vi "Main.vi"(11 "Module Admin":refnum<class "Delacor_lib_QMH_Cloneable Module Admin.lvclass">) -> ()   [LabVIEW 2026, in "UserEventRecorder.lvlib"]
doc: "This template is based off of the Queued Message Handler design pattern and the Queued Message Handler project template that ships with LabVIEW.\n\nThe main difference is that the queue is private to this module and communication between modules is performed via Broadcast and Request events.\n\nRequest events are wrapped in public API methods and are handled in the Event Handling Loop (EHL) of this VI. Any module can register for Broadcast events sent by this module. The EHL generates messages based on user interface actions.\n\nThe Message Handling Loop (MHL) processes messages generated by the EHL, or by other messages. The messages are string values, so new messages can be added easily to the Message Cases case structure in the MHL. Each message cluster can also provide an optional value for Message Data, which is a variant that can be converted to whatever message-specific data is required.\n_____\nBased on DQMH Dev Tools: Project Template 7.1.2.1547."
uses:
  UserEventRecorder.lvlib
  <vilib>/Delacor/Delacor QMH/Libraries/Cloneable Module Admin_class/Delacor_lib_QMH_Cloneable Module Admin.lvclass
  TestEvent.ctl
  <vilib>/Wovalab/Utilities/Helper Loop Periodic Timing/Late Execution Mode--enum.ctl
  KeyboardAndMouseDataAcquisition.ctl
  <vilib>/Wovalab/Utilities/Helper Loop Periodic Timing/Helper Loop Periodic Timing.lvclass/Helper Loop Periodic Timing.ctl
  Module Data--cluster.ctl
  <vilib>/Delacor/Delacor QMH/Libraries/Cloneable Module Admin_class/Delacor_lib_QMH_Cloneable Module Admin.lvclass/Delacor_lib_QMH_Cloneable Module Admin.ctl
  Record Frame Mouse Metadata Argument--cluster.ctl
  <vilib>/Delacor/Delacor QMH/Libraries/Message Queue_class/Delacor_lib_QMH_Message Queue.lvclass/Delacor_lib_QMH_Message Queue.ctl
  Stop Argument--cluster.ctl
  <vilib>/Delacor/Delacor QMH/Libraries/Module Admin_class/Delacor_lib_QMH_Module Admin.lvclass/Delacor_lib_QMH_Module Admin.ctl
  <vilib>/Utility/miscctls.llb/LVPointTypeDef.ctl
  6b0c7d21-e3a6-4e04-8aec-f5c565291270.vi
  7c070138-7b6f-4615-b0c4-f77ec53dd64e.vi
  <vilib>/Delacor/Delacor QMH/Libraries/Cloneable Module Admin_class/Delacor_lib_QMH_Get Module ID.vi
  <vilib>/Wovalab/Utilities/Helper Loop Periodic Timing/Read Current Number Of Execution.vi
  <vilib>/Delacor/Delacor QMH/Libraries/Message Queue_class/Delacor_lib_QMH_Enqueue Message (Single).vi
  <vilib>/Delacor/Delacor QMH/Libraries/Module Admin_class/Delacor_lib_QMH_Get External Launch.vi
  <vilib>/Wovalab/Utilities/Helper Loop Periodic Timing/Stop Helper Loop Internal.vi
  <vilib>/Wovalab/Utilities/Helper Loop Periodic Timing/U32 Max Value--constant.vi
  <vilib>/Wovalab/Utilities/Helper Loop Periodic Timing/Update Last Execution Time.vi
  <vilib>/Wovalab/Utilities/Helper Loop Periodic Timing/Loops Events AE.vi
  <vilib>/Wovalab/Utilities/Helper Loop Periodic Timing/Notify Monitoring Window.vi
  <vilib>/Wovalab/Utilities/Helper Loop Periodic Timing/Monitoring--global.vi
  Core/global.vi
  <userlib>/_OpenG.lib/comparison/comparison.llb/String Changed__ogtk.vi
  <vilib>/Utility/inputDevices.llb/mouseAcquire.vi
  <vilib>/Utility/inputDevices.llb/keyboardAcquire.vi
  <vilib>/JDP Science/JSONtext/Variant to JSON Text.vi
  <vilib>/Utility/inputDevices.llb/closeMouse.vi
  <vilib>/Utility/inputDevices.llb/closeKeyboard.vi
  <vilib>/Wovalab/Utilities/Helper Loop Periodic Timing/Helper Loop Periodic Timing.lvclass
  <vilib>/JDP Science/JSONtext/LVClass Serializer/JSONtext LVClass Serializer.lvclass
  <vilib>/Delacor/Delacor QMH/Libraries/Message Queue_class/Delacor_lib_QMH_Message Queue.lvclass
  Launcher/Launcher.lvlib
  Core/Core.lvlib
  <userlib>/_OpenG.lib/comparison/comparison.llb/openg_comparison__ogtk.lvlib
panel:
  out "TestEvent":T1
  out "axis info":T2
  out "button info":T3
  out "keys pressed":T4(array[ring])
  out "error out":errorcluster
  out "Status":string
  in  "Simulate EHL Error":bool
  in  "Simulate MHL Error":bool
  # "Other processes communicate with this Module via its Public API (wrappers for its Request Events).\n\nThis Module communicates with other processes via its Broadcast Events.\nAny process that wants to receive these messages can register for this module's Broadcast events."
  # "This template is for the DQMH framework. See the block diagram for more information on how to use this template."
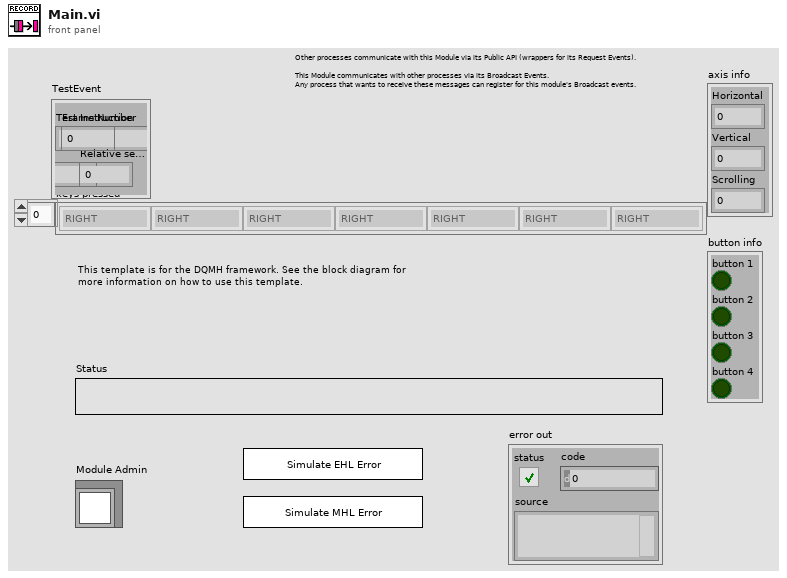
[diagram p1: front panel]
types:
  T1 = typedef "TestEvent.ctl" = cluster{"Test Instruction":string, "Sample Number":u32, "Relative seconds":dbl, "Frame Number":u32}
  T2 = cluster{"Horizontal":i32, "Vertical":i32, "Scrolling":i32}
  T3 = cluster{"button 1":bool, "button 2":bool, "button 3":bool, "button 4":bool}
  T4 = enum16{"0", "1", "2", "3", "4", "5", "6", "7", "8", "9", "A", "B", "C", "D", "E", "F", "G", "H", "I", "J", "K", "L", "M", "N", "O", "P", "Q", "R", "S", "T", "U", "V", "W", "X", "Y", "Z", "F1", "F2", "F3", "F4", "F5", "F6", "F7", "F8", "F9", "F10", "F11", "F12", "F13", "F14", "F15", "ADD", "BACK", "BACKSLASH", "CAPITAL", "COMMA", "DECIMAL", "DELETE", "DIVIDE", "DOWN", "END", "EQUALS", "ESCAPE", "GRAVE (`)", "HOME", "INSERT", "LBRACKET", "LCONTROL", "LEFT", "L ALT", "LSHIFT", "LWIN", "MINUS", "MULTIPLY", "NEXT", "NUMLOCK", "NUMPAD_0", "NUMPAD_1", "NUMPAD_2", "NUMPAD_3", "NUMPAD_4", "NUMPAD_5", "NUMPAD_6", "NUMPAD_7", "NUMPAD_8", "NUMPAD_9", "PAUSE", "PERIOD", "PRIOR (PG UP)", "RBRACKET", "RCONTROL", "RETURN", "RIGHT", "R ALT", "RSHIFT", "RWIN", "SCROLL", "SEMICOLON", "SLASH", "SPACE", "SUBTRACT", "TAB", "UP", "ENTER (num pad)", "' (quote)"}[]
  T5 = typedef "KeyboardAndMouseDataAcquisition.ctl" = cluster{"axis info":cluster{"Horizontal":i32, "Vertical":i32, "Scrolling":i32}, "button info":cluster{"button 1":bool, "button 2":bool, "button 3":bool, "button 4":bool}, "Relative Time (User Event)":dbl, "Sample Number":u32, "Relative Time (Frame 0)":dbl, "key mode":enum16{"RELATIVE", "ABSOLUTE"}, "Frame Number":u32, "Keyboard Key Pressed":enum16{"0", "1", "2", "3", "4", "5", "6", "7", "8", "9", "A", "B", "C", "D", "E", "F", "G", "H", "I", "J", "K", "L", "M", "N", "O", "P", "Q", "R", "S", "T", "U", "V", "W", "X", "Y", "Z", "F1", "F2", "F3", "F4", "F5", "F6", "F7", "F8", "F9", "F10", "F11", "F12", "F13", "F14", "F15", "ADD", "BACK", "BACKSLASH", "CAPITAL", "COMMA", "DECIMAL", "DELETE", "DIVIDE", "DOWN", "END", "EQUALS", "ESCAPE", "GRAVE (`)", "HOME", "INSERT", "LBRACKET", "LCONTROL", "LEFT", "L ALT", "LSHIFT", "LWIN", "MINUS", "MULTIPLY", "NEXT", "NUMLOCK", "NUMPAD_0", "NUMPAD_1", "NUMPAD_2", "NUMPAD_3", "NUMPAD_4", "NUMPAD_5", "NUMPAD_6", "NUMPAD_7", "NUMPAD_8", "NUMPAD_9", "PAUSE", "PERIOD", "PRIOR (PG UP)", "RBRACKET", "RCONTROL", "RETURN", "RIGHT", "R ALT", "RSHIFT", "RWIN", "SCROLL", "SEMICOLON", "SLASH", "SPACE", "SUBTRACT", "TAB", "UP", "ENTER (num pad)", "' (quote)"}, "Keyboard No Op":bool}
  T6 = typedef "Wovalab_lib_Utilities.lvlib/Helper Loop Periodic Timing.lvclass/Late Execution Mode--enum.ctl" = enum16{"No change", "Process missed periods ignoring original phase", "Process missed periods maintaining original phase"}
  T7 = typedef "UserEventRecorder.lvlib/Request Events--cluster.ctl" = cluster{"Stop Module":refnum<user-event>, "Show Panel":refnum<user-event>, "Hide Panel":refnum<user-event>, "Show Diagram":refnum<user-event>, "Get Module Execution Status":refnum<user-event>, "Record Frame Mouse Metadata":refnum<user-event>, "Local Instance":T8}
  T8 = typedef "UserEventRecorder.lvlib/Local Instance Request Events--cluster.ctl" = cluster{"Test Event Triggered":refnum<user-event>}
  T9 = typedef "Launcher.lvlib/Broadcast Events--cluster.ctl" = cluster{"Module Did Init":refnum<user-event>, "Status Updated":refnum<user-event>, "Error Reported":refnum<user-event>, "Module Did Stop":refnum<user-event>, "Update Module Execution Status":refnum<user-event>, "Start Capture Detection Loop":refnum<user-event>, "Benchmark Started":refnum<user-event>, "Broadcast number of frames and run ID":refnum<user-event>}
  T10 = typedef "UserEventRecorder.lvlib/Module Data--cluster.ctl" = cluster{"Status":string}
  T11 = enum16{"0", "1", "2", "3", "4", "5", "6", "7", "8", "9", "A", "B", "C", "D", "E", "F", "G", "H", "I", "J", "K", "L", "M", "N", "O", "P", "Q", "R", "S", "T", "U", "V", "W", "X", "Y", "Z", "F1", "F2", "F3", "F4", "F5", "F6", "F7", "F8", "F9", "F10", "F11", "F12", "F13", "F14", "F15", "ADD", "BACK", "BACKSLASH", "CAPITAL", "COMMA", "DECIMAL", "DELETE", "DIVIDE", "DOWN", "END", "EQUALS", "ESCAPE", "GRAVE (`)", "HOME", "INSERT", "LBRACKET", "LCONTROL", "LEFT", "L ALT", "LSHIFT", "LWIN", "MINUS", "MULTIPLY", "NEXT", "NUMLOCK", "NUMPAD_0", "NUMPAD_1", "NUMPAD_2", "NUMPAD_3", "NUMPAD_4", "NUMPAD_5", "NUMPAD_6", "NUMPAD_7", "NUMPAD_8", "NUMPAD_9", "PAUSE", "PERIOD", "PRIOR (PG UP)", "RBRACKET", "RCONTROL", "RETURN", "RIGHT", "R ALT", "RSHIFT", "RWIN", "SCROLL", "SEMICOLON", "SLASH", "SPACE", "SUBTRACT", "TAB", "UP", "ENTER (num pad)", "' (quote)"}
  T12 = enum32{"invalid lock state", "Not Locked", "Locked (No Password)", "Password-protected"}
  T13 = typedef "UserEventRecorder.lvlib/Stop Argument--cluster.ctl" = cluster{"Module ID":i32, "Origin":string, "Exit via Stop Module Req?":bool, "Wait for Module to stop?":bool}
  T14 = typedef "LVPointTypeDef.ctl" = cluster{"Horizontal":i16, "Vertical":i16}
  T15 = enum32{"Invalid", "Standard", "Closed", "Hidden", "Minimized", "Maximized"}
  T16 = typedef "UserEventRecorder.lvlib/Record Frame Mouse Metadata Argument--cluster.ctl" = cluster{"Module ID":i32, "KeyboardAndMouseData":T5}
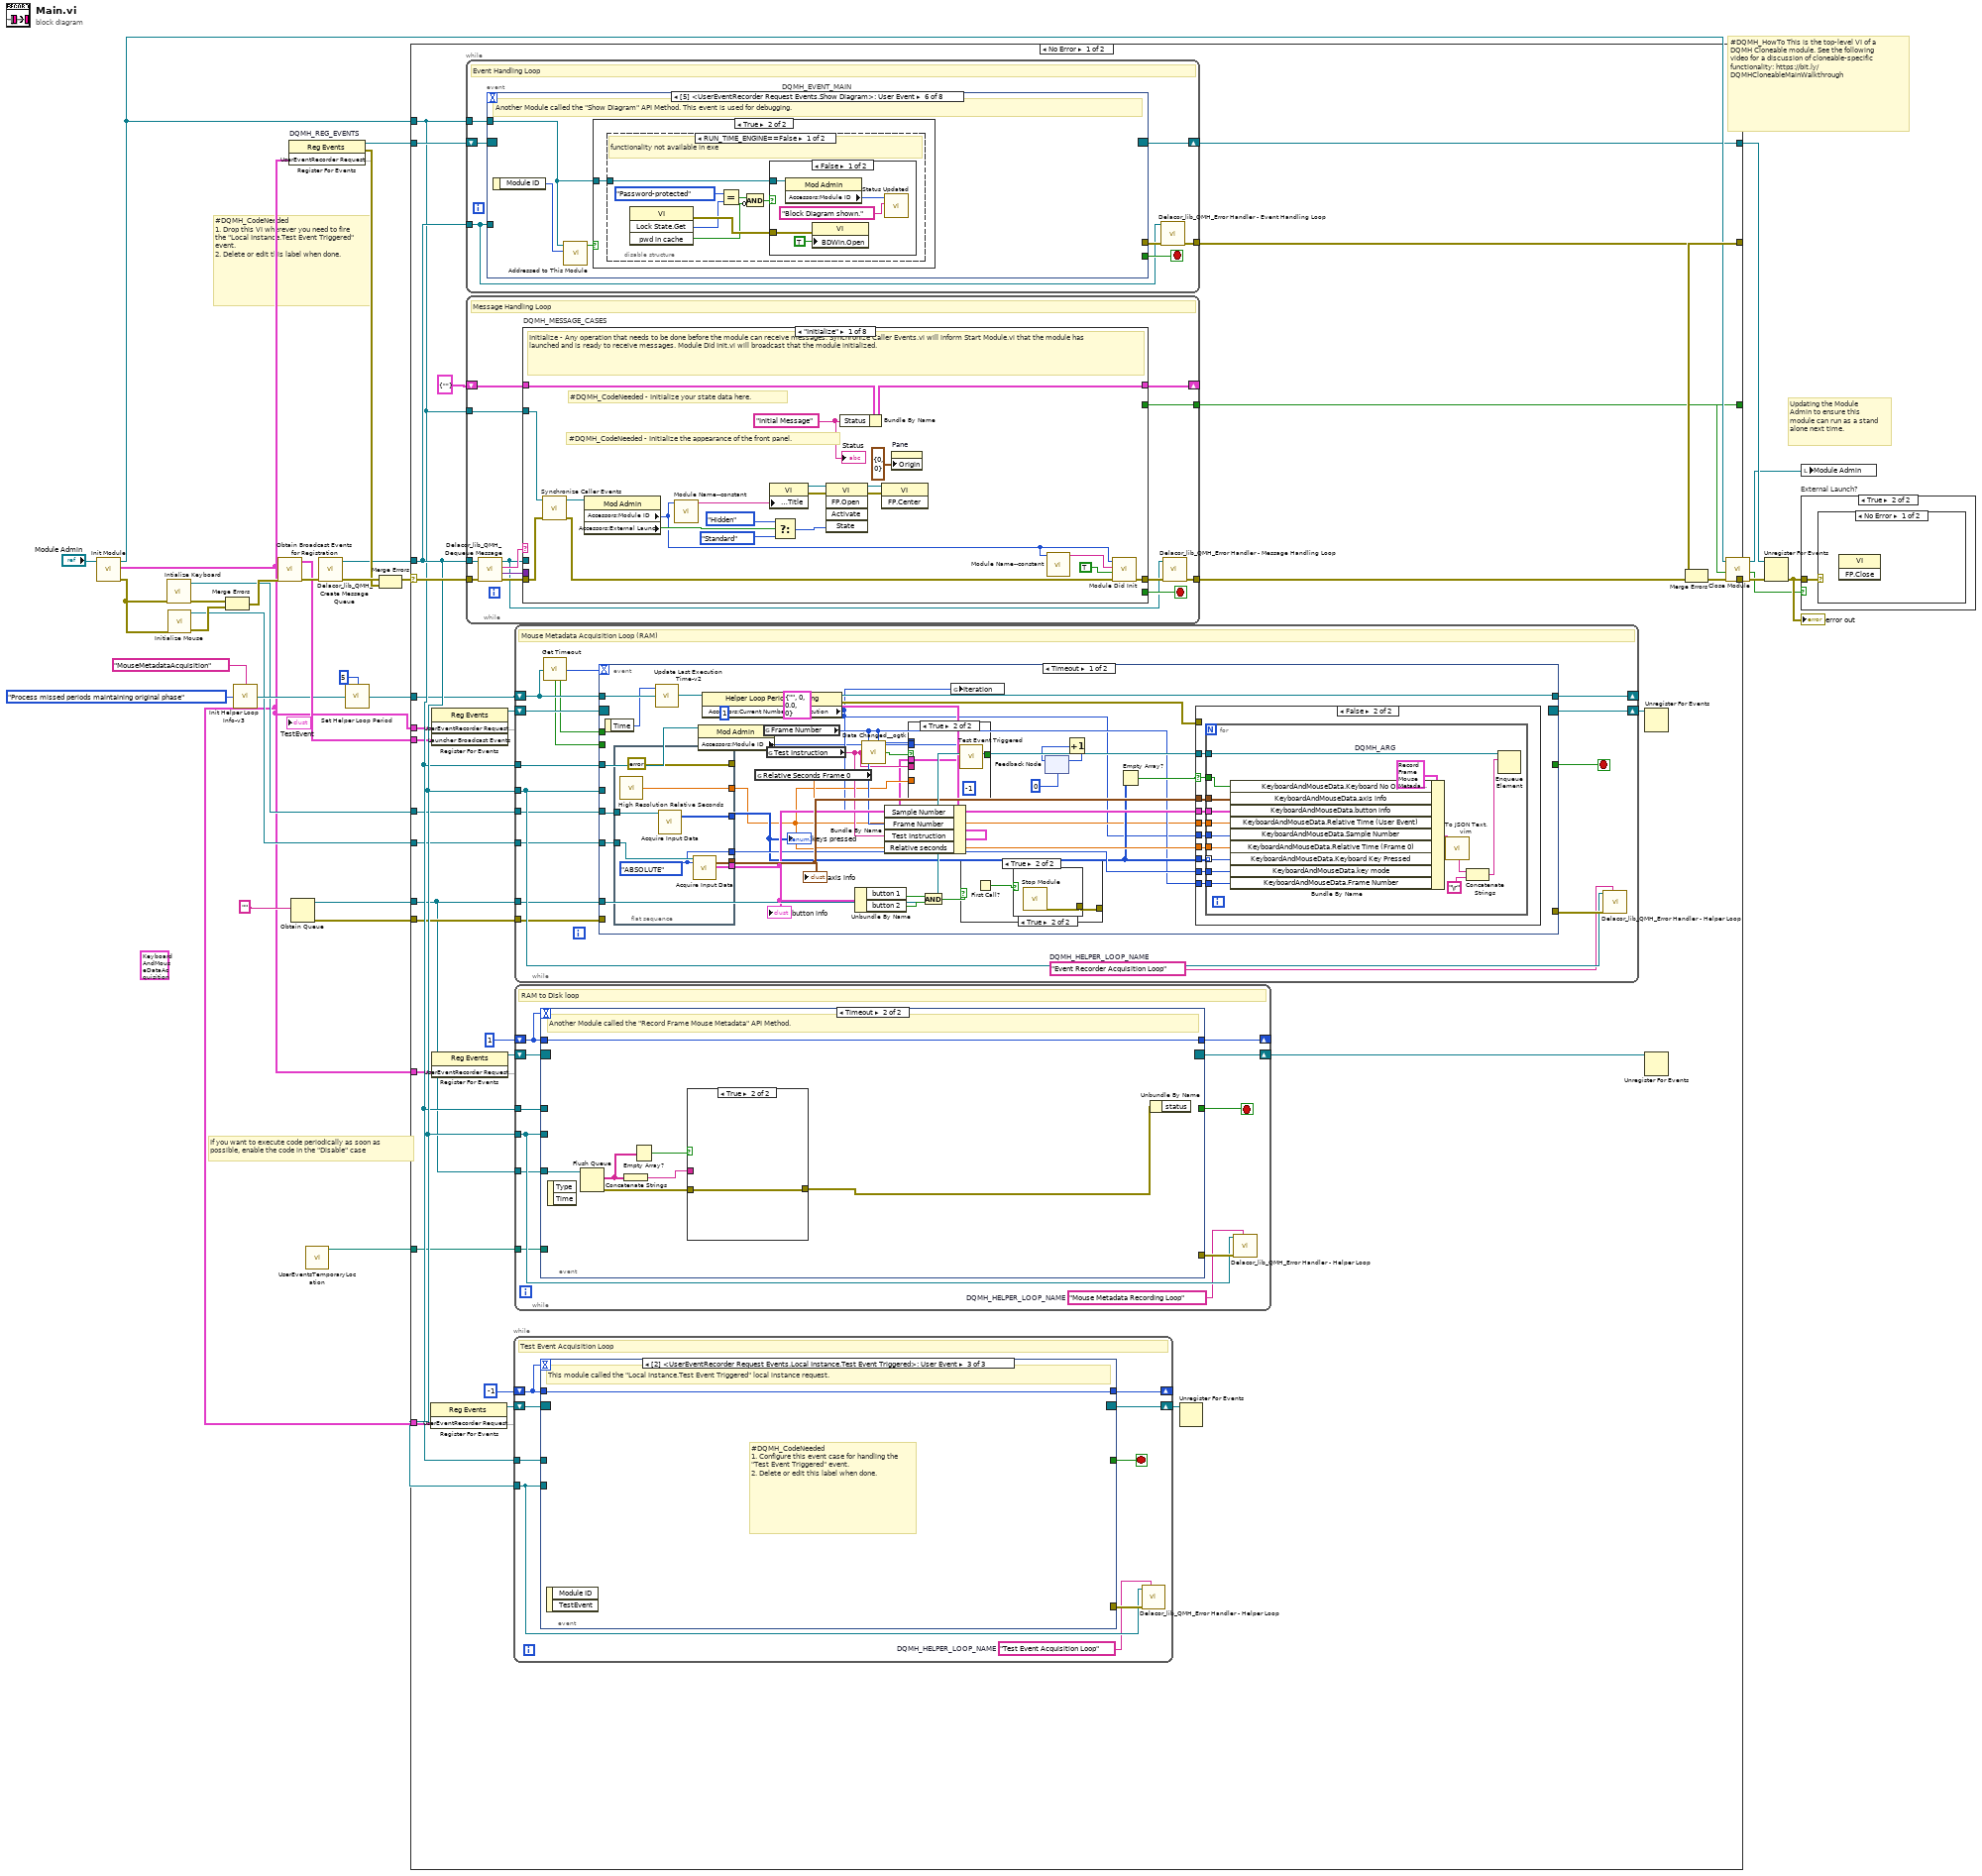
[diagram p0: block diagram]
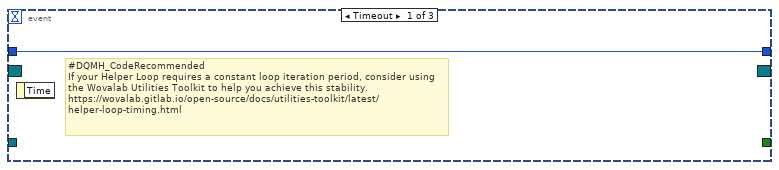
[diagram p2: hidden frame]
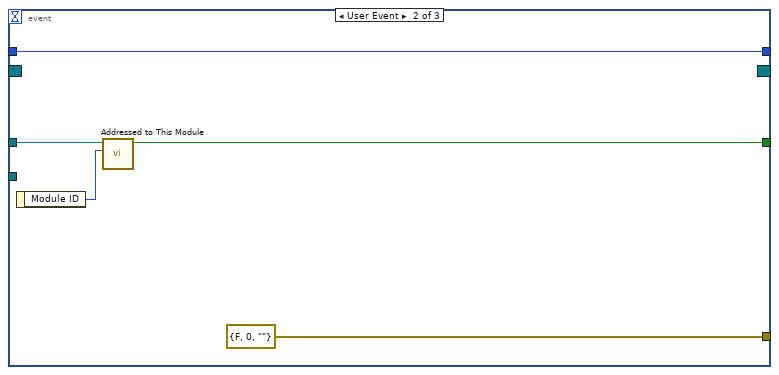
[diagram p3: hidden frame]
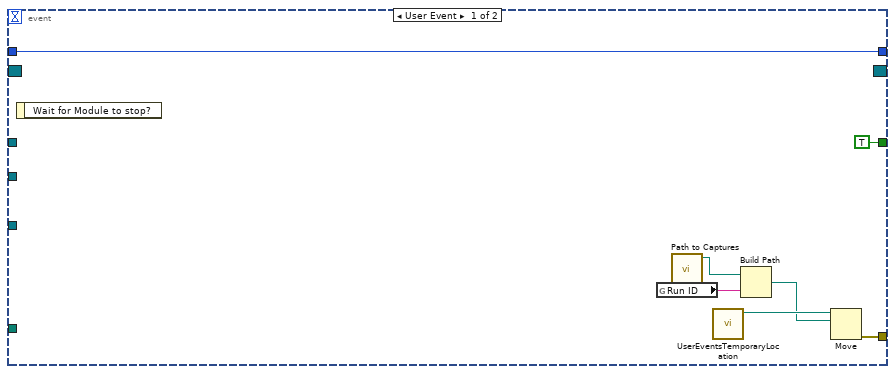
[diagram p4: hidden frame]
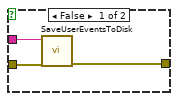
[diagram p5: hidden frame]
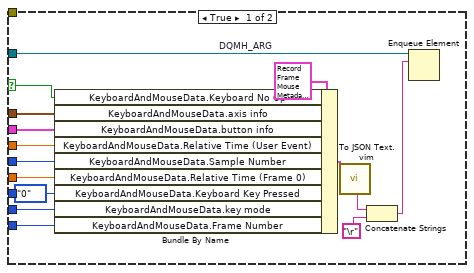
[diagram p7: hidden frame]
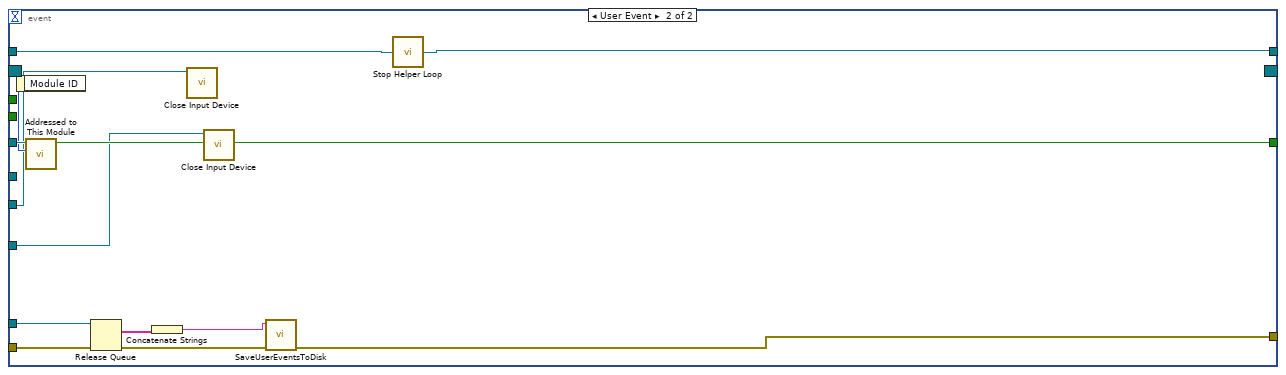
[diagram p10: hidden frame]
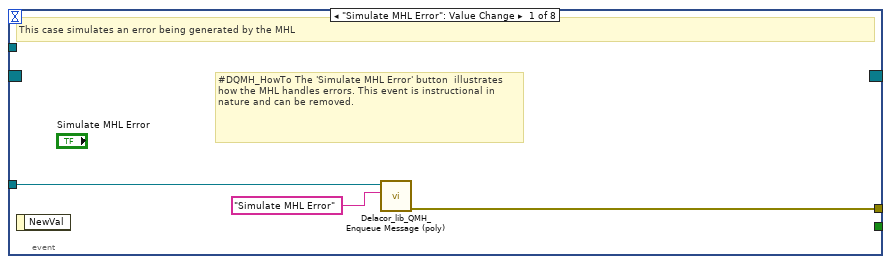
[diagram p11: hidden frame]
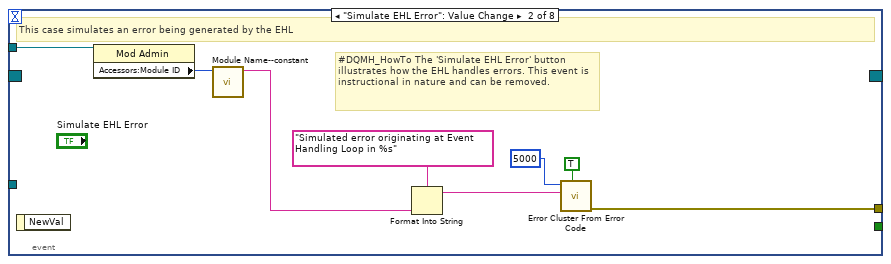
[diagram p12: hidden frame]
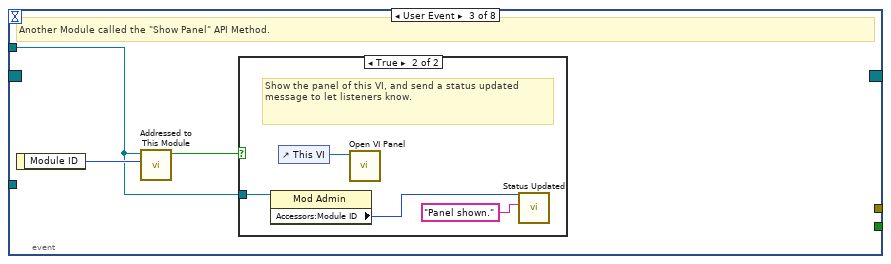
[diagram p13: hidden frame]
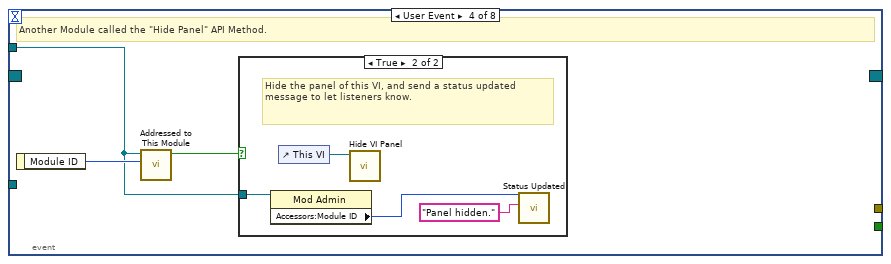
[diagram p15: hidden frame]
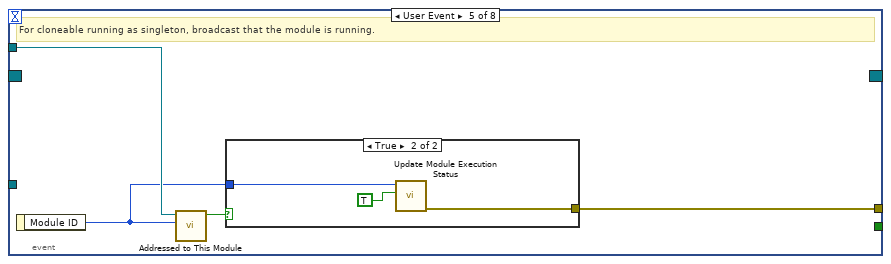
[diagram p17: hidden frame]
diagram:
  (unwired) T5 {"axis info"={"Horizontal"=0, "Vertical"=0, "Scrolling"=0}, "button info"={"button 1"=FALSE, "button 2"=FALSE, "button 3"=FALSE, "button 4"=FALSE}, "Relative Time (User Event)"=0.0, "Sample Number"=0, "Relative Time (Frame 0)"=0.0, "key mode"=enum."ABSOLUTE", "Frame Number"=0, "Keyboard Key Pressed"=enum."RIGHT", "Keyboard No Op"=FALSE} ("KeyboardAndMouseData")
  # "#DQMH_CodeNeeded\n1. Drop this VI wherever you need to fire the \"Local Instance.Test Event Triggered\" event.\n2. Delete or edit this label when done."
  # "If you want to execute code periodically as soon as possible, enable the code in the \"Disable\" case"
  # "#DQMH_HowTo This is the top-level VI of a DQMH Cloneable module. See the following video for a discussion of cloneable-specific functionality: https://bit.ly/DQMHCloneableMainWalkthrough"
  # "Updating the Module Admin to ensure this module can run as a stand alone next time."
  n1 = call "Init Module.vi"("Cloneable Module Admin in"="Module Admin") -> ("error out"=w11:errorcluster, "UserEventRecorder Request Events"=w1:T7, "Cloneable Module Admin out"=w22:refnum<class "Delacor_lib_QMH_Cloneable Module Admin.lvclass">)  [unwired: 8 in]
  n2 = call <vilib>:"Intialize Keyboard.vi"("error in (no error)"=w11) -> ("error out"=w10:errorcluster, "device ID"=w7:refnum<k1>)  [unwired: 9 out]
  n3 = call <vilib>:"Initialize Mouse.vi"("error in (no error)"=w11) -> ("error out"=w9:errorcluster, "device ID"=w6:refnum<k1>)  [unwired: 9 out]
  n4 = Merge Errors(w10, w9) -> (w8:errorcluster)
  n5 = call <vilib>:"Init Helper Loop Info-v3.vi"("Late Execution Mode (Process missed periods ignoring original phase)"=Late_Execution_Mode--enum."Process missed periods maintaining original phase", "Loop Name (\"\": Caller VI)"="MouseMetadataAcquisition" ("Loop Name (\"\": Caller VI)")) -> ("Helper Loop Periodic Timing"=w14:refnum<class "Helper Loop Periodic Timing.lvclass">)
  n6 = call "Obtain Broadcast Events for Registration.vi"("error in"=w8) -> ("error out"=w18:errorcluster, "Launcher Broadcast Events"=w17:T9)  [unwired: 8 in, 1 out]
  n7 = register-events "DQMH_REG_EVENTS"(w1) -> (reference out=w25:refnum<event-registration>, error out=w27:errorcluster)  [unwired: 2 in]
  n8 = Obtain Queue(element data type="") -> (queue out=w3:refnum<queue>, error out=w4:errorcluster)  [unwired: 4 in, 1 out]
  n9 = call "UserEventsTemporaryLocation.vi"() -> ("UserEventsPath"=w12:path)  [unwired: 11 in]
  n10 = call <vilib>:"Delacor_lib_QMH_Create Message Queue.vi"("error in"=w18) -> ("error out"=w29:errorcluster, "Message Queue"=w24:refnum<class "Delacor_lib_QMH_Message Queue.lvclass">)  [unwired: 9 in]
  n11 = call <vilib>:"Set Helper Loop Period.vi"("Period (ms)"=5, "Helper Loop Periodic Timing in"=w14) -> ("Helper Loop Periodic Timing out"=w13:refnum<class "Helper Loop Periodic Timing.lvclass">)  [unwired: 13 in]
  n12 = Merge Errors(w29, w27) -> (w28:errorcluster)
  n13 = case shown="No Error" w28 {
    selector: w28 -> [w59 w418]
    tunnel: [w61 w417] -> w32
    tunnel: [w58 w416] -> w26
    tunnel: w25 -> [w57 w416]
    tunnel: w24 -> [w56 w409]
    tunnel: [w60 _] -> w33
    tunnel: w22 -> [w55 w412]
    tunnel: [w54 _] -> w20
    tunnel: w1 -> [w53 _]
    tunnel: w17 -> [w50 _]
    tunnel: w1 -> [w49 _]
    tunnel: w13 -> [w45 _]
    tunnel: w12 -> [w44 _]
    tunnel: w7 -> [w42 _]
    tunnel: w6 -> [w41 _]
    tunnel: w4 -> [w40 _]
    tunnel: w3 -> [w39 _]
    tunnel: w1 -> [w38 _]
    frame No Error {
      n14 = register-events ("DQMH_HELPER_REGFOREVENTS")(w38) -> (reference out=w36:refnum<event-registration>)  [unwired: 2 in, 1 out]
      n15 = register-events ("DQMH_HELPER_REGFOREVENTS")(w53, w50) -> (reference out=w51:refnum<event-registration>)  [unwired: 2 in, 1 out]
      n16 = register-events ("DQMH_HELPER_REGFOREVENTS")(w49) -> (reference out=w47:refnum<event-registration>)  [unwired: 2 in, 1 out]
      n17 = while {
        tunnel: w56 -> [w219]
        shift-right: [w222] -> w58
        shift-left: w57 -> [w223]
        tunnel: [w224] -> w60
        tunnel: w55 -> [w220]
        stop <- w221 stop-if-true
        # "Event Handling Loop"
        n18 = event "DQMH_EVENT_MAIN" shown="[5] <UserEventRecorder Request Events.Show Diagram>: User Event" {
          selector: w223 -> [_ _ _ _ _ _ _ _]
          dyn-events: [_ _ _ _ _ _ _ _] -> w222
          timeout: _ -> [_ _ _ _ _ _ _ _]
          tunnel: [_ _ _ _ _ _ w277 _] -> w221
          tunnel: w219 -> [w227 _ _ _ _ _ w280 w297]
          tunnel: [w228 w236 _ _ w254 _ w281 w300] -> w225
          tunnel: w220 -> [_ w235 w237 w244 w252 w258 w279 w298]
          event "Simulate MHL Error": Value Change {
            # "#DQMH_HowTo The 'Simulate MHL Error' button  illustrates how the MHL handles errors. This event is instructional in nature and can be removed."
            # "This case simulates an error being generated by the MHL"
            n19 = event-data() -> ()  [unwired: 1 in, 1 out]
            n20 = call-poly <vilib>:"Delacor_lib_QMH_Enqueue Message (poly).vi"("Message"="Simulate MHL Error", "Message Queue in"=w227) -> ("error out"=w228:errorcluster)  [unwired: 8 in, 1 out]
          }
          event "Simulate EHL Error": Value Change {
            # "#DQMH_HowTo The 'Simulate EHL Error' button  illustrates how the EHL handles errors. This event is instructional in nature and can be removed."
            # "This case simulates an error being generated by the EHL"
            n21 = event-data() -> ()  [unwired: 1 in, 1 out]
            n22 = property on="Property Node" class="Mod Admin"(reference=w235) -> ("Accessors:Module ID"=w234:i32)  [unwired: 1 in, 2 out]
            n23 = call "Module Name--constant.vi"("Module ID"=w234) -> ("Module Name"=w229:string)  [unwired: 10 in]
            n24 = Format Into String(format string="Simulated error originating at Event Handling Loop in %s", w229) -> (resulting string=w232:string)  [unwired: 2 in, 1 out]
            n25 = call <vilib>:"Error Cluster From Error Code.vi"("show call chain? (False)"=TRUE, "error message (\"\")"=w232, "error code (0)"=5000) -> ("error out"=w236:errorcluster)  [unwired: 6 in]
          }
          event User Event {
            # "Another Module called the \"Show Panel\" API Method."
            n26 = event-data() -> ("Module ID"=w238:i32)  [unwired: 1 in]
            n27 = call "Addressed to This Module.vi"("Module ID from Argument"=w238, "Module Admin"=w237) -> ("Addressed to this instance?"=w239:bool)  [unwired: 8 in, 1 out]
            n28 = case shown="True" w239 {
              tunnel: w237 -> [_ w241]
              frame False {
              }
              frame True {
                # "Show the panel of this VI, and send a status updated message to let listeners know."
                n29 = property on="Property Node" class="Mod Admin"(reference=w241) -> ("Accessors:Module ID"=w240:i32)  [unwired: 1 in, 2 out]
                n30 = control-ref of="This VI"() -> (w243:refnum<vi>)
                n31 = call "Open VI Panel.vi"("VI"=w243) -> ()  [unwired: 10 in, 1 out]
                n32 = call "Status Updated.vi"("Status"="Panel shown." ("format string"), "Module ID"=w240) -> ()  [unwired: 9 in, 1 out]
              }
            }
          }
          event User Event {
            # "Another Module called the \"Hide Panel\" API Method."
            n33 = event-data() -> ("Module ID"=w245:i32)  [unwired: 1 in]
            n34 = call "Addressed to This Module.vi"("Module ID from Argument"=w245, "Module Admin"=w244) -> ("Addressed to this instance?"=w246:bool)  [unwired: 8 in, 1 out]
            n35 = case shown="True" w246 {
              tunnel: w244 -> [_ w248]
              frame False {
              }
              frame True {
                # "Hide the panel of this VI, and send a status updated message to let listeners know."
                n36 = property on="Property Node" class="Mod Admin"(reference=w248) -> ("Accessors:Module ID"=w247:i32)  [unwired: 1 in, 2 out]
                n37 = control-ref of="This VI"() -> (w250:refnum<vi>)
                n38 = call "Hide VI Panel.vi"("VI"=w250) -> ()  [unwired: 10 in, 1 out]
                n39 = call "Status Updated.vi"("Status"="Panel hidden." ("format string"), "Module ID"=w247) -> ()  [unwired: 9 in, 1 out]
              }
            }
          }
          event User Event {
            # "For cloneable running as singleton, broadcast that the module is running."
            n40 = event-data() -> ("Module ID"=w251:i32)  [unwired: 1 in]
            n41 = call "Addressed to This Module.vi"("Module ID from Argument"=w251, "Module Admin"=w252) -> ("Addressed to this instance?"=w253:bool)  [unwired: 8 in, 1 out]
            n42 = case shown="True" w253 {
              tunnel: [_ w257] -> w254
              tunnel: w251 -> [_ w256]
              frame False {
              }
              frame True {
                n43 = call "Update Module Execution Status.vi"("Running?"=TRUE, "Module ID"=w256) -> ("error out"=w257:errorcluster)  [unwired: 9 in]
              }
            }
          }
          event User Event {
            # "Another Module called the \"Show Diagram\" API Method. This event is used for debugging."
            n44 = event-data() -> ("Module ID"=w259:i32)  [unwired: 1 in]
            n45 = call "Addressed to This Module.vi"("Module ID from Argument"=w259, "Module Admin"=w258) -> ("Addressed to this instance?"=w260:bool)  [unwired: 8 in, 1 out]
            n46 = case shown="True" w260 {
              tunnel: w258 -> [_ w261]
              frame False {
              }
              frame True {
                n47 = disable-structure shown="RUN_TIME_ENGINE==False" {
                  disable-tunnel: w261 -> [w262 _]
                  frame condition #0 (active) {
                    # "functionality not available in exe"
                    n48 = invoke on="Invoke Node" class="VI" method="Lock State.Get"() -> (error out=w268:errorcluster, "Get Lock State"=w267:T12, "pwd in cache"=w264:bool)  [unwired: 4 in, 1 out]
                    n49 = Equal?(x=T12."Password-protected", y=w267) -> (x = y?=w265:bool)
                    n50 = Compound Arithmetic op=AND(w265, invert w264) -> (w263:bool)
                    n51 = case shown="False" w263 {
                      tunnel: w268 -> [w273 _]
                      tunnel: w262 -> [w270 _]
                      frame False {
                        n52 = property on="Property Node" class="Mod Admin"(reference=w270) -> ("Accessors:Module ID"=w269:i32)  [unwired: 1 in, 2 out]
                        n53 = property on="Property Node" class="VI"(error in=w273, "BDWin.Open"=TRUE ("Block Diagram Window:Open")) -> ()  [unwired: 1 in, 2 out]
                        n54 = call "Status Updated.vi"("Status"="Block Diagram shown." ("format string"), "Module ID"=w269) -> ()  [unwired: 9 in, 1 out]
                      }
                      frame True {
                        # "Password-protected VI, and the password is not in the cache. Do not show the diagram."
                      }
                    }
                  }
                  frame condition #1 {
                  }
                }
              }
            }
          }
          event User Event {
            # "Another Module called the \"Stop Module\" API Method  or the Message Handling Loop below."
            n55 = event-data() -> ("Module ID"=w275:i32, "Wait for Module to stop?"=w276:bool, "Origin"=w274:string)  [unwired: 1 in]
            n56 = call "Addressed to This Module.vi"("Module ID from Argument"=w275, "Module Admin"=w279) -> ("Addressed to this instance?"=w278:bool)  [unwired: 8 in, 1 out]
            n57 = case shown="True" w278 {
              tunnel: [_ w293] -> w281
              tunnel: w280 -> [_ w289]
              tunnel: [_ TRUE] -> w277
              tunnel: w276 -> [_ w284]
              tunnel: w275 -> [_ w286]
              tunnel: w274 -> [_ w282]
              frame False {
              }
              frame True {
                # "The event can get fired from the Exit message. The queue gets destroyed there. In this case, the Enqueue VI will return error 1. It is safe to ignore, because the module is already exiting."
                n58 = local write "Status"(w282) -> ()
                n59 = Bundle By Name(cluster=T13 {"Module ID"=-1, "Origin"="", "Exit via Stop Module Req?"=FALSE, "Wait for Module to stop?"=FALSE} ("Stop Argument"), "Module ID"=w286, "Exit via Stop Module Req?"=TRUE, "Wait for Module to stop?"=w284) -> (w283:T13)
                n60 = call-poly <vilib>:"Delacor_lib_QMH_Enqueue Message (poly).vi"("Priority Message? (F)"=TRUE, "Message Data"=w283, "Message"="Exit", "Message Queue in"=w289) -> ("error out"=w294:errorcluster)  [unwired: 6 in, 1 out]
                n61 = call <vilib>:"Clear Errors.vi"("error in (no error)"=w294, "specific error code to clear (0: all)"=1) -> ("error out"=w293:errorcluster)  [unwired: 4 in, 1 out]
              }
            }
          }
          event Panel Close? {
            w299 = TRUE  # Discard the event, the MHL is responsible for closing and stopping this VI.
            # "Hide the panel or send the 'Exit' message if the user clicks the 'X' on the module main VI panel."
            n62 = event-data() -> ()  [unwired: 1 in, 1 out]
            n63 = property on="Property Node" class="Mod Admin"(reference=w298) -> (reference out=w295:refnum<class "Delacor_lib_QMH_Cloneable Module Admin.lvclass">, "Accessors:External Launch"=w296:bool)  [unwired: 1 in, 1 out]
            n64 = case shown="True" w296 {
              tunnel: w297 -> [_ w308]
              tunnel: [_ w309] -> w300
              tunnel: w295 -> [w303 _]
              frame True {
                # "If externally launched, clicking the 'X' hides the panel, but doesn't close it."
                n65 = property on="Property Node" class="Mod Admin"(reference=w303) -> ("Accessors:Module ID"=w302:i32)  [unwired: 1 in, 2 out]
                n66 = call "Status Updated.vi"("Status"="Panel hidden." ("format string"), "Module ID"=w302) -> ("error out"=w301:errorcluster)  [unwired: 9 in]
                n67 = control-ref of="This VI"() -> (w305:refnum<vi>)
                n68 = call "Hide VI Panel.vi"("error in"=w301, "VI"=w305) -> ()  [unwired: 9 in, 1 out]
              }
              frame False {
                # "If run as a stand-alone VI, clicking the panel 'X' stops the VI."
                n69 = call-poly <vilib>:"Delacor_lib_QMH_Enqueue Message (poly).vi"("Priority Message? (F)"=TRUE, "Message"="Exit", "Message Queue in"=w308) -> ("error out"=w309:errorcluster)  [unwired: 7 in, 1 out]
              }
            }
            n70 = event-data ("Event Filter Node")("Discard?"=w299) -> ()  [unwired: 1 in, 1 out]
          }
        }
        n71 = call-dynamic "Delacor_lib_QMH_Error Handler - Event Handling Loop.vi"("error in"=w225, "Message Queue in"=w219) -> ("dup error in"=w224:errorcluster)  [unwired: 8 in, 1 out]
      }
      n72 = while {
        tunnel: w56 -> [w310]
        shift-right: [w317] -> _
        shift-left: T10 {"Status"=""} ("Data Cluster") -> [w318]
        tunnel: w59 -> [w321]
        tunnel: [w319] -> w61
        tunnel: w55 -> [w312]
        tunnel: [w311] -> w54
        stop <- w316 stop-if-true
        # "Message Handling Loop"
        n73 = call-dynamic "Delacor_lib_QMH_Dequeue Message.vi"("error in"=w321, "Message Queue in"=w310) -> ("error out"=w320:errorcluster, "Message Data"=w314:variant, "Message"=w315:string, "Message Queue out"=w313:refnum<class "Delacor_lib_QMH_Message Queue.lvclass">)  [unwired: 6 in]
        n74 = case "DQMH_MESSAGE_CASES" shown="\"Initialize\"" w315 {
          selector: w315 -> [_ _ _ _ _ _ _ w398]
          tunnel: w313 -> [_ _ _ _ w353 _ w390 _]
          tunnel: w320 -> [w341 w345 w348 w350 w362 w379 w396 w407]
          tunnel: [w339 w345 w347 w350 w358 w378 w391 w408] -> w322
          tunnel: w318 -> [w332 w344 w346 w349 w357 w376 w389 w405]
          tunnel: [w331 w344 w346 w349 w357 w376 w389 w405] -> w317
          tunnel: [_ _ _ _ _ _ w388 _] -> w316
          tunnel: w314 -> [_ _ _ _ w356 _ w386 _]
          tunnel: w312 -> [w327 _ _ _ w355 w374 w381 w404]
          tunnel: [_ _ _ _ _ _ w384 _] -> w311
          frame "Initialize" {
            w324 = "Initial Message" ("Initial Message")
            # "#DQMH_CodeNeeded - Initialize the appearance of the front panel."
            # "#DQMH_CodeNeeded - Initialize your state data here."
            # "Initialize - Any operation that needs to be done before the module can receive messages. Synchronize Caller Events.vi will inform Start Module.vi that the module has launched and is ready to receive messages. Module Did Init.vi will broadcast that the module initialized."
            n75 = call "Synchronize Caller Events.vi"("error in"=w341, "Module Admin"=w327) -> ("error out"=w340:errorcluster, "Module Admin out"=w326:refnum<class "Delacor_lib_QMH_Cloneable Module Admin.lvclass">)  [unwired: 8 in]
            n76 = property on="Property Node" class="Mod Admin"(reference=w326) -> ("Accessors:Module ID"=w323:i32, "Accessors:External Launch"=w328:bool)  [unwired: 1 in, 2 out]
            n77 = call "Module Name--constant.vi"("Module ID"=w323) -> ("Module Name"=w336:string)  [unwired: 10 in]
            n78 = property on="Property Node" class="VI"("Front Panel.Title"=w336) -> (reference out=w338:refnum<vi>, error out=w343:errorcluster)  [unwired: 2 in]
            n79 = Select(t=T15."Hidden" ("State"), s=w328, f=T15."Standard" ("State")) -> (s? t:f=w333:T15)
            n80 = invoke on="Invoke Node" class="VI" method="FP.Open"(reference=w338, error in=w343, "State"=w333) -> (reference out=w337:refnum<vi>, error out=w342:errorcluster)  [unwired: 2 in, 3 out]
            n81 = Bundle By Name(cluster=w332, "Status"=w324) -> (w331:T10)
            n82 = invoke on="Invoke Node" class="VI" method="FP.Center"(reference=w337, error in=w342) -> ()  [unwired: 1 in, 3 out]
            n83 = property on="Pane" class="Pane"("Origin"=T14 {"Horizontal"=0, "Vertical"=0}) -> ()  [unwired: 2 in, 2 out]
            n84 = call "Module Name--constant.vi"("Module ID"=w323) -> ("Module Name"=w329:string)  [unwired: 10 in]
            n85 = call "Module Did Init.vi"("error in"=w340, "Initialized?"=TRUE, "Origin"=w329, "Module ID"=w323) -> ("error out"=w339:errorcluster)  [unwired: 7 in]
            "Status" <- w324
          }
          frame "---Module Specific---" {
            # "Separator -- The following cases handle messages specific to this Module."
          }
          frame "---Copy This Frame---" {
            # "Duplicate this frame when creating new messages.  Change this comment in the duplicated frame to describe this message."
            n86 = Merge Errors(w348) -> (w347:errorcluster)
          }
          frame "---Exit and Error Handling---" {
            # "Separator - the following cases handle errors and exit messages."
          }
          frame "Error" {
            # "#DQMH_CodeRecommended - If the module is running in standalone mode (External Launch = FALSE), this code will pop up an error dialog and call the 'Exit' message if an error occurs. Add more fine-grained error management here."
            # "Error - Check the error message data and respond accordingly. This message is sent by the \"Error Handler\" VIs at the end of each loop in this application."
            n87 = property on="Property Node" class="Mod Admin"(reference=w355) -> ("Accessors:External Launch"=w354:bool, "Accessors:Module ID"=w352:i32)  [unwired: 1 in, 2 out]
            n88 = Variant To Data(error in=w362, type=errorcluster {"status"=FALSE, "code"=0, "source"=""} ("error constant"), Variant=w356) -> (data=w351:errorcluster, error out=w360:errorcluster)
            n89 = local write "error out"(w351) -> ()
            n90 = call "Error Reported.vi"("Error"=w351, "Module ID"=w352) -> ()  [unwired: 9 in, 1 out]
            n91 = case shown="False" w354 {
              tunnel: [w367 _] -> w359
              tunnel: w353 -> [w365 _]
              tunnel: w351 -> [w366 _]
              frame False {
                n92 = disable-structure shown="Default" {
                  disable-tunnel: w366 -> [w368 _]
                  frame condition #0 (active) {
                    # "If the module is running standalone, then pop up an error dialog and call the \"Exit\" message."
                    n93 = call <vilib>:"Simple Error Handler.vi"("error in (no error)"=w368) -> ()  [unwired: 4 in, 5 out]
                  }
                  frame condition #1 {
                    # "To prevent the Simple Error Handler VI from being loaded (e.g. when deploying to a Real-Time target), add the Conditional Disable Symbol \"DQMH_Disable_SEH\" to your project and set it to TRUE."
                  }
                }
                n94 = call-poly <vilib>:"Delacor_lib_QMH_Enqueue Message (poly).vi"("Priority Message? (F)"=TRUE, "Message"="Exit", "Message Queue in"=w365) -> ("error out"=w367:errorcluster)  [unwired: 7 in, 1 out]
              }
              frame True {
                # "If the module was launched externally, calling the Error Reported broadcast VI is the only action performed by the \"Error\" message. The module's caller can then process the error appropriately."
              }
            }
            n95 = Merge Errors(w360, w359) -> (w358:errorcluster)
          }
          frame "Simulate MHL Error" {
            # "#DQMH_HowTo The 'Simulate MHL Error' button  illustrates how the MHL handles errors. This event is instructional in nature and can be removed."
            # "Simulate an error occurring at the MHL"
            n96 = property on="Property Node" class="Mod Admin"(reference=w374) -> ("Accessors:Module ID"=w375:i32)  [unwired: 1 in, 2 out]
            n97 = call "Module Name--constant.vi"("Module ID"=w375) -> ("Module Name"=w370:string)  [unwired: 10 in]
            n98 = Format Into String(format string="Simulated error originating at Message Handling Loop in %s", w370) -> (resulting string=w371:string)  [unwired: 2 in, 1 out]
            n99 = call <vilib>:"Error Cluster From Error Code.vi"("show call chain? (False)"=TRUE, "error message (\"\")"=w371, "error code (0)"=5001) -> ("error out"=w377:errorcluster)  [unwired: 6 in]
            n100 = Merge Errors(w379, w377) -> (w378:errorcluster)
          }
          frame "Exit" {
            w387 = 91  # 91: not all Exit messages will have an argument
            w388 = TRUE  # Stop the VI
            # "Release the message queue reference"
            # "#DQMH_CodeNeeded - Add any required cleanup code here."
            # "Exit - Exit the application."
            n101 = Variant To Data(error in=w396, type=T13 {"Module ID"=-1, "Origin"="", "Exit via Stop Module Req?"=FALSE, "Wait for Module to stop?"=FALSE} ("Stop Argument"), Variant=w386) -> (data=w383:T13, error out=w392:errorcluster)
            n102 = call <vilib>:"Clear Errors.vi"("error in (no error)"=w392, "specific error code to clear (0: all)"=w387) -> ("error out"=w395:errorcluster)  [unwired: 4 in, 1 out]
            n103 = property on="Property Node" class="Mod Admin"(reference=w381) -> ("Accessors:Module ID"=w380:i32)  [unwired: 1 in, 2 out]
            n104 = control-ref of="This VI"() -> (w382:refnum<vi>)
            n105 = call-dynamic "Delacor_lib_QMH_Release Message Queue.vi"("error in"=w395, "Message Queue"=w390) -> ("error out"=w394:errorcluster)  [unwired: 9 in]
            n106 = call "Handle Exit.vi"("Stop Argument"=w383, "Module Admin in"=w381, "VI reference"=w382) -> ("error out"=w393:errorcluster, "Wait for Stop?"=w384:bool)  [unwired: 7 in]
            n107 = Merge Errors(w394, w393) -> (w391:errorcluster)
            n108 = call "Error Reported.vi"("Error"=w391, "Module ID"=w380) -> ()  [unwired: 9 in, 1 out]
          }
          frame Default {
            # "'Default' case only runs if there is a message that isn't defined in any of the other cases.  Output a programming error."
            n109 = property on="Property Node" class="Mod Admin"(reference=w404) -> ("Accessors:Module ID"=w403:i32)  [unwired: 1 in, 2 out]
            n110 = call "Module Name--constant.vi"("Module ID"=w403) -> ("Module Name"=w397:string)  [unwired: 10 in]
            n111 = Format Into String(format string="The invalid message string \"%s\" was received in the Message Handling Loop for module \"%s\".", w398, w397) -> (resulting string=w400:string)  [unwired: 2 in, 1 out]
            n112 = call <vilib>:"Error Cluster From Error Code.vi"("show call chain? (False)"=TRUE, "error message (\"\")"=w400, "error code (0)"=1) -> ("error out"=w406:errorcluster)  [unwired: 6 in]
            n113 = Merge Errors(w407, w406) -> (w408:errorcluster)
          }
        }
        n114 = call-dynamic "Delacor_lib_QMH_Error Handler - Message Handling Loop.vi"("error in"=w322, "Message Queue in"=w313) -> ("dup error in"=w319:errorcluster)  [unwired: 8 in, 1 out]
      }
      n115 = while "DQMH_HELPER_LOOP" {
        shift-right: [w70] -> _
        shift-left: -1 -> [w69]
        shift-right: [w67] -> w37
        shift-left: w36 -> [w68]
        tunnel: w56 -> [w64]
        tunnel: w55 -> [w62]
        stop <- w66 stop-if-true
        w63 = "Test Event Acquisition Loop"  # DQMH_HELPER_LOOP_NAME
        # "Test Event Acquisition Loop"
        n116 = event "DQMH_HELPER_EVENT_STRUCTURE" shown="[2] <UserEventRecorder Request Events.Local Instance.Test Event Triggered>: User Event" {
          selector: w68 -> [_ _ _]
          dyn-events: [_ _ _] -> w67
          timeout: w69 -> [_ _ _]
          tunnel: w69 -> [w71 w76 w77]
          tunnel: [w71 w76 w77] -> w70
          tunnel: [_ w73 _] -> w66
          tunnel: [_ errorcluster {"status"=FALSE, "code"=0, "source"=""} ("error constant") _] -> w65
          tunnel: w64 -> [_ _ _]
          tunnel: w62 -> [_ w74 _]
          event Timeout {
            # "#DQMH_CodeRecommended\nIf your Helper Loop requires a constant loop iteration period, consider using the Wovalab Utilities Toolkit to help you achieve this stability.\nhttps://wovalab.gitlab.io/open-source/docs/utilities-toolkit/latest/helper-loop-timing.html"
            n117 = event-data() -> ()  [unwired: 1 in, 1 out]
          }
          event User Event {
            n118 = event-data() -> ("Module ID"=w72:i32)  [unwired: 1 in]
            n119 = call "Addressed to This Module.vi"("Module ID from Argument"=w72, "Module Admin"=w74) -> ("Addressed to this instance?"=w73:bool)  [unwired: 8 in, 1 out]
          }
          event User Event {
            # "#DQMH_CodeNeeded\n1. Configure this event case for handling the \"Test Event Triggered\" event.\n2. Delete or edit this label when done."
            # "This module called the \"Local Instance.Test Event Triggered\" local instance request."
            n120 = event-data() -> ()  [unwired: 1 in, 2 out]
          }
        }
        n121 = call-dynamic "Delacor_lib_QMH_Error Handler - Helper Loop.vi"("Error Debug"=w63, "error in"=w65, "Message Queue in"=w64) -> ()  [unwired: 7 in, 2 out]
      }
      n122 = while "DQMH_HELPER_LOOP" {
        shift-right: [w122] -> _
        shift-left: w45 -> [w114]
        shift-right: [w120] -> w52
        shift-left: w51 -> [w121]
        tunnel: w56 -> [w117]
        tunnel: w55 -> [w115]
        tunnel: w42 -> [w110]
        tunnel: w41 -> [w109]
        tunnel: w40 -> [w108]
        tunnel: w39 -> [w107]
        stop <- w119 stop-if-true
        w116 = "Event Recorder Acquisition Loop"  # DQMH_HELPER_LOOP_NAME
        # "Mouse Metadata Acquisition Loop (RAM)"
        n123 = call <vilib>:"Get Timeout.vi"("Helper Loop Periodic Timing"=w114) -> ("Timeout (ms)"=w113:i32, "Late?"=w112:bool, "First Execution Since Period Modification?"=w111:bool)  [unwired: 12 in]
        n124 = event "DQMH_HELPER_EVENT_STRUCTURE" shown="[0] Timeout" {
          selector: w121 -> [_ _]
          dyn-events: [_ _] -> w120
          timeout: w113 -> [_ _]
          tunnel: w114 -> [w149 w215]
          tunnel: [w133 w214] -> w122
          tunnel: [_ w217] -> w119
          tunnel: [_ w206] -> w118
          tunnel: w117 -> [_ _]
          tunnel: w115 -> [w124 w218]
          tunnel: w112 -> [_ _]
          tunnel: w111 -> [_ _]
          tunnel: w110 -> [w147 w213]
          tunnel: w109 -> [w146 w212]
          tunnel: w108 -> [_ w210]
          tunnel: w107 -> [w142 w211]
          event Timeout {
            (unwired) -1 ("Module ID")
            (unwired) i16 1 ("vKey")
            n125 = event-data() -> ("Time"=w148:u32)  [unwired: 1 in]
            n126 = flat-sequence {
              tunnel: [w205] -> w127
              tunnel: [errorcluster {"status"=FALSE, "code"=0, "source"=""} ("error out")] -> _
              tunnel: w147 -> [w203]
              tunnel: w146 -> [w202]
              tunnel: [w201] -> w136
              tunnel: [w200] -> w141
              tunnel: [w199] -> w140
              tunnel: [w198] -> w138
              frame #0 {
                w198 = enum16{"RELATIVE", "ABSOLUTE"}."ABSOLUTE" ("key mode")
                n127 = call <vilib>:"High Resolution Relative Seconds.vi"() -> ("relative seconds"=w205:dbl)
                n128 = call-poly <vilib>:"Acquire Input Data.vi"("device ID"=w203) -> ("keys pressed"=w201:T4)  [unwired: 1 in, 17 out]
                n129 = call-poly <vilib>:"Acquire Input Data.vi"("device ID"=w202, "key mode"=w198) -> ("axis info"=w200:T2, "button info"=w199:T3)  [unwired: 1 in, 15 out]
              }
            }
            n130 = call <vilib>:"Update Last Execution Time-v2.vi"("Time"=w148, "Helper Loop Periodic Timing in"=w149) -> ("Helper Loop Periodic Timing out"=w134:refnum<class "Helper Loop Periodic Timing.lvclass">)  [unwired: 12 in, 1 out]
            n131 = property class="Mod Admin"(reference=w124) -> ("Accessors:Module ID"=w123:i32)  [unwired: 1 in, 2 out]
            n132 = property class="Helper Loop Periodic Timing"(reference=w134) -> (reference out=w133:refnum<class "Helper Loop Periodic Timing.lvclass">, error out=w132:errorcluster, "Accessors:Current Number Of Execution"=w125:u64)  [unwired: 1 in]
            n133 = global read "global.vi" "Relative Seconds Frame 0"() -> (w139:dbl)
            n134 = global read "global.vi" "Frame Number"() -> (w129:u32)
            n135 = global read "global.vi" "Test Instruction"() -> (w128:string)
            n136 = Unbundle By Name(w140) -> ("button 1"=w145:bool, "button 2"=w144:bool)
            n137 = call-poly <userlib>:"Data Changed__ogtk.vi"("String"=w128) -> ("Changed"=w131:bool)
            n138 = Bundle By Name(cluster=T1 {"Test Instruction"="", "Sample Number"=0, "Relative seconds"=0.0, "Frame Number"=0} ("TestEvent"), "Sample Number"=w125, "Frame Number"=w129, "Test Instruction"=w128, "Relative seconds"=w127) -> (w126:T1)
            n139 = case shown="True" w131 {
              selector: w131 -> [w152 _]
              tunnel: w129 -> [_ _]
              tunnel: w128 -> [_ _]
              tunnel: w127 -> [_ _]
              tunnel: w126 -> [_ w154]
              tunnel: [w152 _] -> _
              tunnel: w123 -> [_ w153]
              frame False {
              }
              frame True {
                n140 = call "Test Event Triggered.vi"("TestEvent"=w154, "Module ID"=w153) -> ()  [unwired: 9 in, 1 out]
              }
            }
            n141 = And(x=w145, y=w144) -> (x .and. y?=w143:bool)
            n142 = global write "global.vi" "Iteration"(w125) -> ()
            n143 = case shown="True" w143 {
              tunnel: [_ w196] -> _
              frame False {
              }
              frame True {
                n144 = First Call?() -> (First Call?: T/F=w195:bool)
                n145 = case shown="True" w195 {
                  tunnel: [_ w197] -> w196
                  frame False {
                  }
                  frame True {
                    n146 = call "Stop Module.vi"() -> ("error out"=w197:errorcluster)  [unwired: 11 in]
                  }
                }
              }
            }
            n147 = feedback #1(u32 0 ("Frame Number")) -> (w137:u32)
            n148 = Increment(x=w137) -> (x+1=w150:u32)
            n149 = feedback-in #1(w150) -> ()
            n150 = Empty Array?(array=w136) -> (empty?=w135:bool)
            n151 = case shown="False" w135 {
              selector: w135 -> [w155 w170]
              tunnel: w142 -> [w169 w179]
              tunnel: w141 -> [w168 w178]
              tunnel: w140 -> [w167 w177]
              tunnel: w127 -> [w166 w176]
              tunnel: w139 -> [w165 w175]
              tunnel: w129 -> [w164 w174]
              tunnel: w138 -> [w163 w173]
              tunnel: w125 -> [w162 w172]
              tunnel: w136 -> [_ w171]
              tunnel: w132 -> [_ _]
              frame True {
                w161 = T16 {"Module ID"=-1, "KeyboardAndMouseData"={"axis info"={"Horizontal"=0, "Vertical"=0, "Scrolling"=0}, "button info"={"button 1"=FALSE, "button 2"=FALSE, "button 3"=FALSE, "button 4"=FALSE}, "Relative Time (User Event)"=0.0, "Sample Number"=0, "Relative Time (Frame 0)"=0.0, "key mode"=enum."ABSOLUTE", "Frame Number"=0, "Keyboard Key Pressed"=enum."RIGHT", "Keyboard No Op"=FALSE}}  # DQMH_ARG
                n152 = Bundle By Name(cluster=w161, "KeyboardAndMouseData.Keyboard No Op"=w155, "KeyboardAndMouseData.axis info"=w168, "KeyboardAndMouseData.button info"=w167, "KeyboardAndMouseData.Relative Time (User Event)"=w166, "KeyboardAndMouseData.Sample Number"=w162, "KeyboardAndMouseData.Relative Time (Frame 0)"=w165, "KeyboardAndMouseData.Keyboard Key Pressed"=T11."0", "KeyboardAndMouseData.key mode"=w163, "KeyboardAndMouseData.Frame Number"=w164) -> (w160:T16)
                n153 = call "To JSON Text.vim"("Anything"=w160) -> ("<JSON>"=w158:string)  [unwired: 9 in, 1 out]
                n154 = Concatenate Strings(w158, "\r") -> (w157:string)
                n155 = Enqueue Element(queue=w169, element=w157) -> ()  [unwired: 2 in, 3 out]
              }
              frame False {
                n156 = for {
                  tunnel: w179 -> [w194]
                  tunnel: w178 -> [w192]
                  tunnel: w177 -> [w191]
                  tunnel: w176 -> [w190]
                  tunnel: w175 -> [w189]
                  tunnel: w171 -> [w188] mode=indexing
                  tunnel: w174 -> [w187]
                  tunnel: w173 -> [w182]
                  tunnel: w172 -> [w181]
                  tunnel: w170 -> [w180]
                  w193 = T16 {"Module ID"=-1, "KeyboardAndMouseData"={"axis info"={"Horizontal"=0, "Vertical"=0, "Scrolling"=0}, "button info"={"button 1"=FALSE, "button 2"=FALSE, "button 3"=FALSE, "button 4"=FALSE}, "Relative Time (User Event)"=0.0, "Sample Number"=0, "Relative Time (Frame 0)"=0.0, "key mode"=enum."ABSOLUTE", "Frame Number"=0, "Keyboard Key Pressed"=enum."RIGHT", "Keyboard No Op"=FALSE}}  # DQMH_ARG
                  n157 = Bundle By Name(cluster=w193, "KeyboardAndMouseData.Keyboard No Op"=w180, "KeyboardAndMouseData.axis info"=w192, "KeyboardAndMouseData.button info"=w191, "KeyboardAndMouseData.Relative Time (User Event)"=w190, "KeyboardAndMouseData.Sample Number"=w181, "KeyboardAndMouseData.Relative Time (Frame 0)"=w189, "KeyboardAndMouseData.Keyboard Key Pressed"=w188, "KeyboardAndMouseData.key mode"=w182, "KeyboardAndMouseData.Frame Number"=w187) -> (w186:T16)
                  n158 = call "To JSON Text.vim"("Anything"=w186) -> ("<JSON>"=w184:string)  [unwired: 9 in, 1 out]
                  n159 = Concatenate Strings(w184, "\r") -> (w183:string)
                  n160 = Enqueue Element(queue=w194, element=w183) -> ()  [unwired: 2 in, 3 out]
                }
              }
            }
            "keys pressed" <- w136
            "button info" <- w140
            "axis info" <- w141
          }
          event User Event {
            n161 = event-data() -> ("Module ID"=w216:i32)  [unwired: 1 in]
            n162 = call "Addressed to This Module.vi"("Module ID from Argument"=w216, "Module Admin"=w218) -> ("Addressed to this instance?"=w217:bool)  [unwired: 8 in, 1 out]
            n163 = Release Queue(queue=w211, error in (no error)=w210) -> (remaining elements=w208:string[], error out=w209:errorcluster)  [unwired: 1 in, 1 out]
            n164 = Concatenate Strings(w208) -> (w207:string)
            n165 = call-poly <vilib>:"Close Input Device.vi"("device ID"=w213) -> ()  [unwired: 1 in, 9 out]
            n166 = call-poly <vilib>:"Close Input Device.vi"("device ID"=w212) -> ()  [unwired: 1 in, 9 out]
            n167 = call "SaveUserEventsToDisk.vi"("error in"=w209, "concatenated string"=w207) -> ("error out"=w206:errorcluster)  [unwired: 9 in]
            n168 = call <vilib>:"Stop Helper Loop.vi"("Helper Loop Periodic Timing in"=w215) -> ("Helper Loop Periodic Timing out"=w214:refnum<class "Helper Loop Periodic Timing.lvclass">)
          }
        }
        n169 = call-dynamic "Delacor_lib_QMH_Error Handler - Helper Loop.vi"("Error Debug"=w116, "error in"=w118, "Message Queue in"=w117) -> ()  [unwired: 7 in, 2 out]
      }
      n170 = while "DQMH_HELPER_LOOP" {
        shift-right: [w88] -> _
        shift-left: 1 -> [w87]
        shift-right: [w85] -> w48
        shift-left: w47 -> [w86]
        tunnel: w56 -> [w82]
        tunnel: w55 -> [w80]
        tunnel: w44 -> [w79]
        tunnel: w39 -> [w78]
        stop <- w84 stop-if-true
        w81 = "Mouse Metadata Recording Loop"  # DQMH_HELPER_LOOP_NAME
        # "RAM to Disk loop"
        n171 = event "DQMH_HELPER_EVENT_STRUCTURE" shown="[1] Timeout" {
          selector: w86 -> [_ _]
          dyn-events: [_ _] -> w85
          timeout: w87 -> [_ _]
          tunnel: w87 -> [w95 w102]
          tunnel: [w95 w102] -> w88
          tunnel: [TRUE _] -> w84
          tunnel: [w89 _] -> w83
          tunnel: w82 -> [_ _]
          tunnel: w80 -> [_ _]
          tunnel: w79 -> [_ _]
          tunnel: w78 -> [_ w101]
          event User Event {
            n172 = event-data() -> ()  [unwired: 1 in, 1 out]
            n173 = global read "global.vi" "Run ID"() -> (w90:string)
            n174 = call "Path to Captures.vi"() -> ("Captures"=w93:path)  [unwired: 11 in]
            n175 = call "UserEventsTemporaryLocation.vi"() -> ("UserEventsPath"=w92:path)  [unwired: 11 in]
            n176 = Build Path(base path=w93, name or relative path=w90) -> (appended path=w91:path)
            n177 = Move(source path=w92, 10:w91) -> (error out=w89:errorcluster)  [unwired: 3 in, 2 out]
          }
          event Timeout {
            # "Another Module called the \"Record Frame Mouse Metadata\" API Method."
            n178 = event-data() -> ()  [unwired: 1 in, 2 out]
            n179 = Flush Queue(queue=w101) -> (remaining elements=w97:string[], error out=w100:errorcluster)  [unwired: 1 in, 1 out]
            n180 = Concatenate Strings(w97) -> (w99:string)
            n181 = Empty Array?(array=w97) -> (empty?=w96:bool)
            n182 = case shown="True" w96 {
              tunnel: w100 -> [w105 w106]
              tunnel: w99 -> [w104 _]
              tunnel: [w103 w106] -> w98
              frame False {
                n183 = call "SaveUserEventsToDisk.vi"("error in"=w105, "concatenated string"=w104) -> ("error out"=w103:errorcluster)  [unwired: 9 in]
              }
              frame True {
              }
            }
            n184 = Unbundle By Name(w98) -> ()  [unwired: 1 out]
          }
        }
        n185 = call-dynamic "Delacor_lib_QMH_Error Handler - Helper Loop.vi"("Error Debug"=w81, "error in"=w83, "Message Queue in"=w82) -> ()  [unwired: 7 in, 2 out]
      }
      n186 = Unregister For Events(event registration refnum=w37) -> ()  [unwired: 1 in, 1 out]
      n187 = Unregister For Events(event registration refnum=w52) -> ()  [unwired: 1 in, 1 out]
      n188 = Unregister For Events(event registration refnum=w48) -> ()  [unwired: 1 in, 1 out]
    }
    frame Error {
      n189 = call "Synchronize Caller Events.vi"("Module Admin"=w412) -> ("Module Admin out"=w411:refnum<class "Delacor_lib_QMH_Cloneable Module Admin.lvclass">)  [unwired: 9 in, 1 out]
      n190 = property on="Property Node" class="Mod Admin"(reference=w411) -> ("Accessors:Module ID"=w410:i32)  [unwired: 1 in, 2 out]
      n191 = call-dynamic "Delacor_lib_QMH_Release Message Queue.vi"("error in"=w418, "Message Queue"=w409) -> ("error out"=w417:errorcluster)  [unwired: 9 in]
      n192 = call "Module Name--constant.vi"("Module ID"=w410) -> ("Module Name"=w415:string)  [unwired: 10 in]
      n193 = Format Into String(format string="An error occurred during initialization. %s is no longer running.", w415) -> (resulting string=w413:string)  [unwired: 2 in, 1 out]
      n194 = call "Error Reported.vi"("Additional Information"=w413, "Error"=w417, "Module ID"=w410) -> ()  [unwired: 8 in, 1 out]
    }
  }
  n195 = Merge Errors(w33, w32) -> (w34:errorcluster)
  n196 = call "Close Module.vi"("error in"=w34, "Wait for stop?"=w20, "Module Admin in"=w22) -> ("error out"=w31:errorcluster, "External Launch"=w19:bool, "Module Admin out"=w21:refnum<class "Delacor_lib_QMH_Cloneable Module Admin.lvclass">)  [unwired: 6 in]
  n197 = Unregister For Events(event registration refnum=w26, error in=w31) -> (error out=w30:errorcluster)
  "error out" <- w30
  n198 = case "External Launch?" shown="True" w19 {
    tunnel: w30 -> [_ w419]
    frame False {
    }
    frame True {
      n199 = case shown="No Error" w419 {
        frame No Error {
          n200 = invoke class="VI" method="FP.Close"() -> ()  [unwired: 3 in, 3 out]
        }
        frame Error {
          n201 = disable-structure shown="Default" {
            frame condition #0 (active) {
              n202 = invoke class="VI" method="FP.Open"("Activate"=TRUE ("Activate?")) -> ()  [unwired: 4 in, 5 out]
            }
            frame condition #1 {
              # "Don't show panel on error if running inside a built EXE."
            }
          }
        }
      }
    }
  }
  n203 = local write "Module Admin"(w21) -> ()
